vi "Withdraw.vi"(6 "wait for reply (T)":bool=TRUE, 7 "Amount":dbl, 8 "error in":errorcluster, 9 "Account Number":string, 10 "Accounts File":path) -> (0 "error out":errorcluster, 1 "timed out?":bool, 2 "New Balance":dbl, 3 "Success":bool)   [LabVIEW 2026, in "Account Manager.lvlib"]
doc: "Withdraws an amount from an account if funds suffice and returns the new balance.\n\n_____\nCreated using DQMH Framework: Event Scripter 7.1.2.1547."
uses:
  Account Manager.lvlib
  Withdraw Argument--cluster.ctl
  Withdraw (Reply Payload)--cluster.ctl
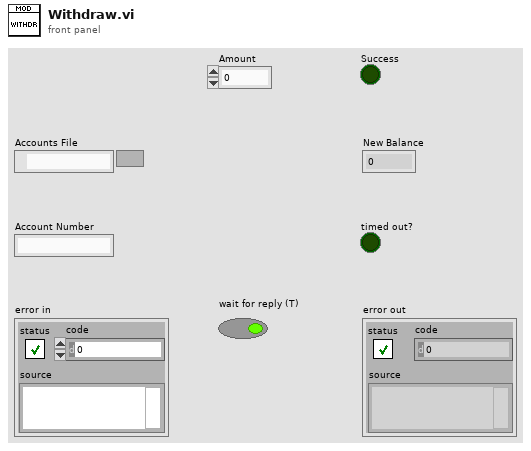
[diagram p1: front panel]
types:
  T1 = typedef "Account Manager.lvlib/Withdraw Argument--cluster.ctl" = cluster{"Accounts File":path, "Account Number":string, "Amount":dbl, "Wait Notifier":refnum<notifier>, "wait for reply":bool}
  T2 = typedef "Account Manager.lvlib/Request Events--cluster.ctl" = cluster{"Stop Module":refnum<user-event>, "Show Panel":refnum<user-event>, "Hide Panel":refnum<user-event>, "Get Module Execution Status":refnum<user-event>, "Show Diagram":refnum<user-event>, "Verify Account":refnum<user-event>, "Get Balance":refnum<user-event>, "Deposit":refnum<user-event>, "Withdraw":refnum<user-event>}
  T3 = typedef "Account Manager.lvlib/Withdraw (Reply Payload)--cluster.ctl" = cluster{"Success":bool, "New Balance":dbl, "error":errorcluster}
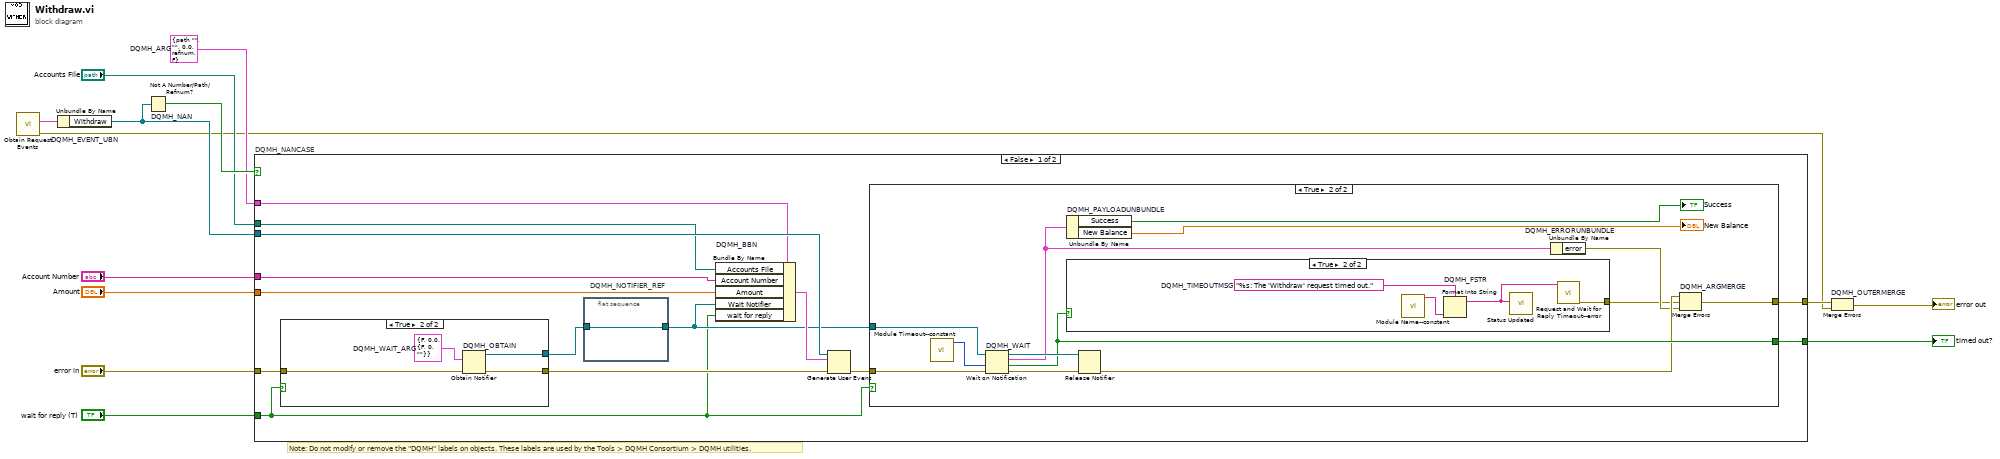
[diagram p0: block diagram]
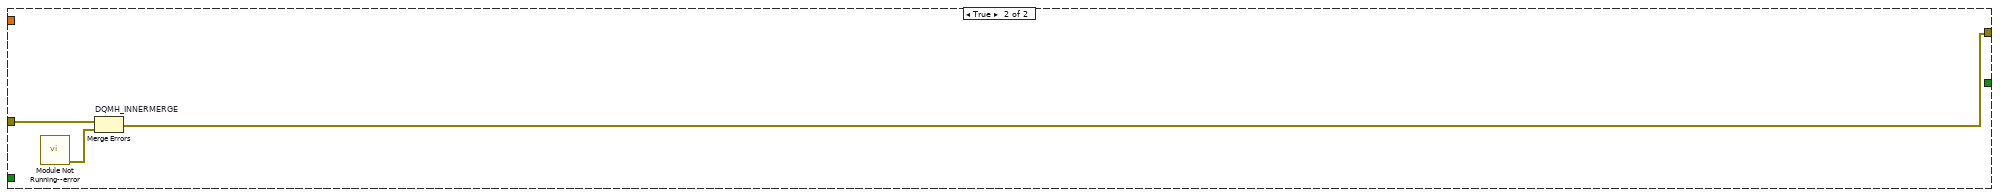
[diagram p5: hidden frame]
diagram:
  w7 = T1 {"Accounts File"=path "", "Account Number"="", "Amount"=0.0, "Wait Notifier"=refnum, "wait for reply"=FALSE}  # DQMH_ARG
  # "Note: Do not modify or remove the \"DQMH\" labels on objects. These labels are used by the Tools > DQMH Consortium > DQMH utilities."
  n1 = call "Obtain Request Events.vi"() -> ("error out"=w2:errorcluster, "Account Manager Request Events"=w1:T2)  [unwired: 10 in]
  n2 = Unbundle By Name "DQMH_EVENT_UBN"(w1) -> ("Withdraw"=w11:refnum<user-event>)
  n3 = Not A Number/Path/Refnum? "DQMH_NAN"(number/path/refnum=w11) -> (NaN/Path/Refnum?=w10:bool)
  n4 = case "DQMH_NANCASE" shown="False" w10 {
    tunnel: "error in" -> [w27 w54]
    tunnel: w11 -> [w25 _]
    tunnel: [w22 w53] -> w8
    tunnel: [w23 _] -> w9
    tunnel: w7 -> [w18 _]
    tunnel: "Accounts File" -> [w17 _]
    tunnel: "Account Number" -> [w16 _]
    tunnel: "Amount" -> [w15 _]
    tunnel: "wait for reply (T)" -> [w14 _]
    frame False {
      n5 = case shown="True" w14 {
        tunnel: w27 -> [w47 w51]
        tunnel: [w47 w50] -> w24
        tunnel: [_ w48] -> w20
        frame False {
        }
        frame True {
          w49 = T3 {"Success"=FALSE, "New Balance"=0.0, "error"={"status"=FALSE, "code"=0, "source"=""}}  # DQMH_WAIT_ARG
          n6 = Obtain Notifier "DQMH_OBTAIN"(notification data type=w49, error in (no error)=w51) -> (notifier out=w48:refnum<notifier>, error out=w50:errorcluster)  [unwired: 2 in, 1 out]
        }
      }
      n7 = flat-sequence "DQMH_NOTIFIER_REF" {
        tunnel: w20 -> [w28]
        tunnel: [w28] -> w19
        frame #0 {
        }
      }
      n8 = Bundle By Name "DQMH_BBN"(cluster=w18, "Accounts File"=w17, "Account Number"=w16, "Amount"=w15, "Wait Notifier"=w19, "wait for reply"=w14) -> (w21:T1)
      n9 = Generate User Event(user event=w25, event data cluster=w21, error in=w24) -> (error out=w26:errorcluster)  [unwired: 1 in, 1 out]
      n10 = case shown="True" w14 {
        tunnel: w26 -> [w29 w42]
        tunnel: w19 -> [_ w41]
        tunnel: [_ w39] -> w23
        tunnel: [w29 w38] -> w22
        frame False {
        }
        frame True {
          n11 = call "Module Timeout--constant.vi"() -> ("Module Timeout"=w32:i32)  [unwired: 11 in]
          n12 = Wait on Notification "DQMH_WAIT"(notifier=w41, timeout in ms (-1)=w32, error in (no error)=w42) -> (notifier out=w40:refnum<notifier>, notification=w33:T3, timed out?=w39:bool, error out=w37:errorcluster)  [unwired: 1 in]
          n13 = Unbundle By Name "DQMH_PAYLOADUNBUNDLE"(w33) -> ("Success"=→"Success":bool, "New Balance"=→"New Balance":dbl)
          n14 = case shown="True" w39 {
            tunnel: [_ w44] -> w34
            frame False {
            }
            frame True {
              w46 = "%s: The 'Withdraw' request timed out."  # DQMH_TIMEOUTMSG
              n15 = call "Module Name--constant.vi"() -> ("Module Name"=w43:string)  [unwired: 11 in]
              n16 = Format Into String "DQMH_FSTR"(format string=w46, w43) -> (resulting string=w45:string)  [unwired: 2 in, 1 out]
              n17 = call "Status Updated.vi"("Status"=w45) -> ()  [unwired: 10 in, 1 out]
              n18 = call "Request and Wait for Reply Timeout--error.vi"("Error Message"=w45) -> ("error out"=w44:errorcluster)  [unwired: 10 in]
            }
          }
          n19 = Release Notifier(notifier=w40, error in (no error)=w37) -> (error out=w36:errorcluster)  [unwired: 1 in, 2 out]
          n20 = Unbundle By Name "DQMH_ERRORUNBUNDLE"(w33) -> ("error"=w35:errorcluster)
          n21 = Merge Errors "DQMH_ARGMERGE"(w36, w34, w35) -> (w38:errorcluster)
        }
      }
    }
    frame True {
      n22 = call "Module Not Running--error.vi"() -> ("error out"=w52:errorcluster)  [unwired: 11 in]
      n23 = Merge Errors "DQMH_INNERMERGE"(w54, w52) -> (w53:errorcluster)
    }
  }
  "timed out?" <- w9
  n24 = Merge Errors "DQMH_OUTERMERGE"(w8, w2) -> (→"error out":errorcluster)
